vi "VIH HelpGen - HTML - Build A HREF Tag to Website.vi"(7 "Escape Reserved HTML chars in body (F)":bool, 11 "URL":string) -> (3 "HTML tag":string)   [LabVIEW 2014]
doc: "::: VI Helpeks :::\nCopyright (c) 2000-2026 Konstantin Shifershteyn. All rights reserved."
panel:
  # "VI Helpeks\nCopyright (c) 2012-2026 Konstantin Shifershteyn"
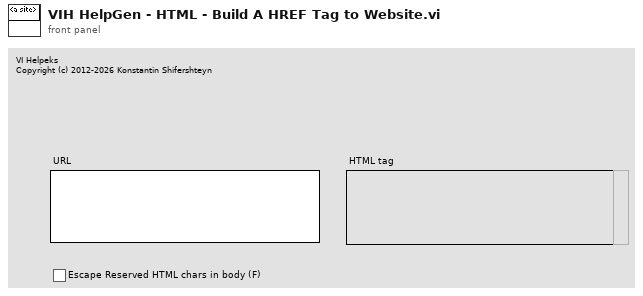
[diagram p1: front panel]
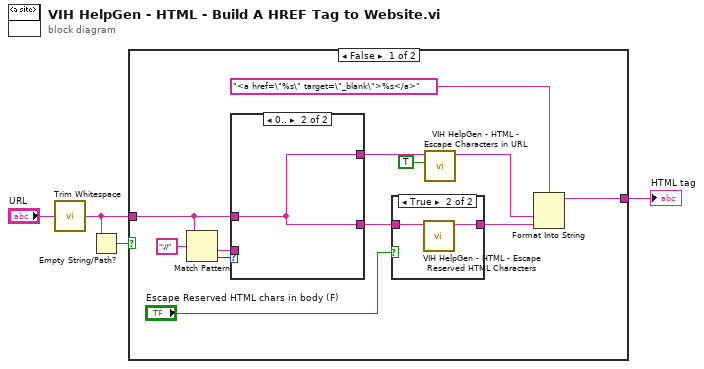
[diagram p0: block diagram]
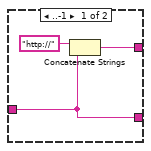
[diagram p3: hidden frame]
diagram:
  n1 = call <vilib>:"Trim Whitespace.vi"("string"="URL") -> ("trimmed string"=w1:string)  [unwired: 1 in]
  n2 = Empty String/Path?(string/path=w1) -> (empty?=w2:bool)
  n3 = case shown="False" w2 {
    tunnel: [w12 w24] -> w4
    tunnel: w1 -> [w11 w24]
    frame False {
      n4 = Match Pattern(string=w11, regular expression="://") -> (after substring=w16:string, offset past match=w15:i32)  [unwired: 1 in, 2 out]
      n5 = case shown="0.." w15 {
        tunnel: w11 -> [w22 w23]
        tunnel: [w21 w23] -> w10
        tunnel: w16 -> [_ _]
        tunnel: [w22 w23] -> w7
        frame ..-1 {
          n6 = Concatenate Strings("http://" ("string"), w22) -> (w21:string)
        }
        frame 0.. {
        }
      }
      n7 = case shown="True" "Escape Reserved HTML chars in body (F)" {
        tunnel: w7 -> [w17 w19]
        tunnel: [w17 w18] -> w6
        frame False {
        }
        frame True {
          n8 = call "VIH HelpGen - HTML - Escape Reserved HTML Characters.vi"("string"=w19) -> ("HTML string"=w18:string)  [unwired: 10 in]
        }
      }
      n9 = call "VIH HelpGen - HTML - Escape Characters in URL.vi"("Escape HTML Reserved chars (T)"=TRUE ("Escape HTML Reserved chars (F)"), "string"=w10) -> ("URL string"=w9:string)  [unwired: 9 in]
      n10 = Format Into String(format string="<a href=\"%s\" target=\"_blank\">%s</a>", w9, w6) -> (resulting string=w12:string)  [unwired: 2 in, 1 out]
    }
    frame True {
    }
  }
  "HTML tag" <- w4
